vi "BSM Burst table save.vi"(6 "SN [ratio]":T1, 7 "Ex info":T4, 8 "error in":errorcluster caption="エラー入力", 9 "BC1":cluster{"B region#":i32, "Date":string}, 10 "BS Path":T2, 11 "Table CP":T3) -> (0 "error out":errorcluster caption="エラー出力", 2 "Table Tag":T5, 3 "Table CV":T6)   [LabVIEW 2018]
panel:
  out "SN":string[](array[string])
  out "Mx Intensity level [pA]":dbl
  out "BL Level [pA]":dbl
  out "Signal Intensity [pA]":dbl
  out "S/N ratio":dbl
  out "BS_E Time Table Path":path
  out "BS_E Signal Table Path":path
  out "BS_E CP Table Path":path
  out "Signal Tag":string[](array[string])
  out "Time Profile A Table":string[][](table) caption="Time A Table"
  out "CP Profile A Table":string[][](table) caption="CP A Table"
  out "Signal Profile A Table":string[][](table) caption="S Table"
  out "サブセット削除後の配列":string[](array[string])
  out "Level Composition":string[](array[string])
  out "Base Ex info array":string[](array[string])
  out "Time Profile Table":string[][](table) caption="Time Table"
  out "CP Profile Table":string[][](table) caption="CP Table"
  out "Signal Profile Table":string[][](table) caption="S Table"
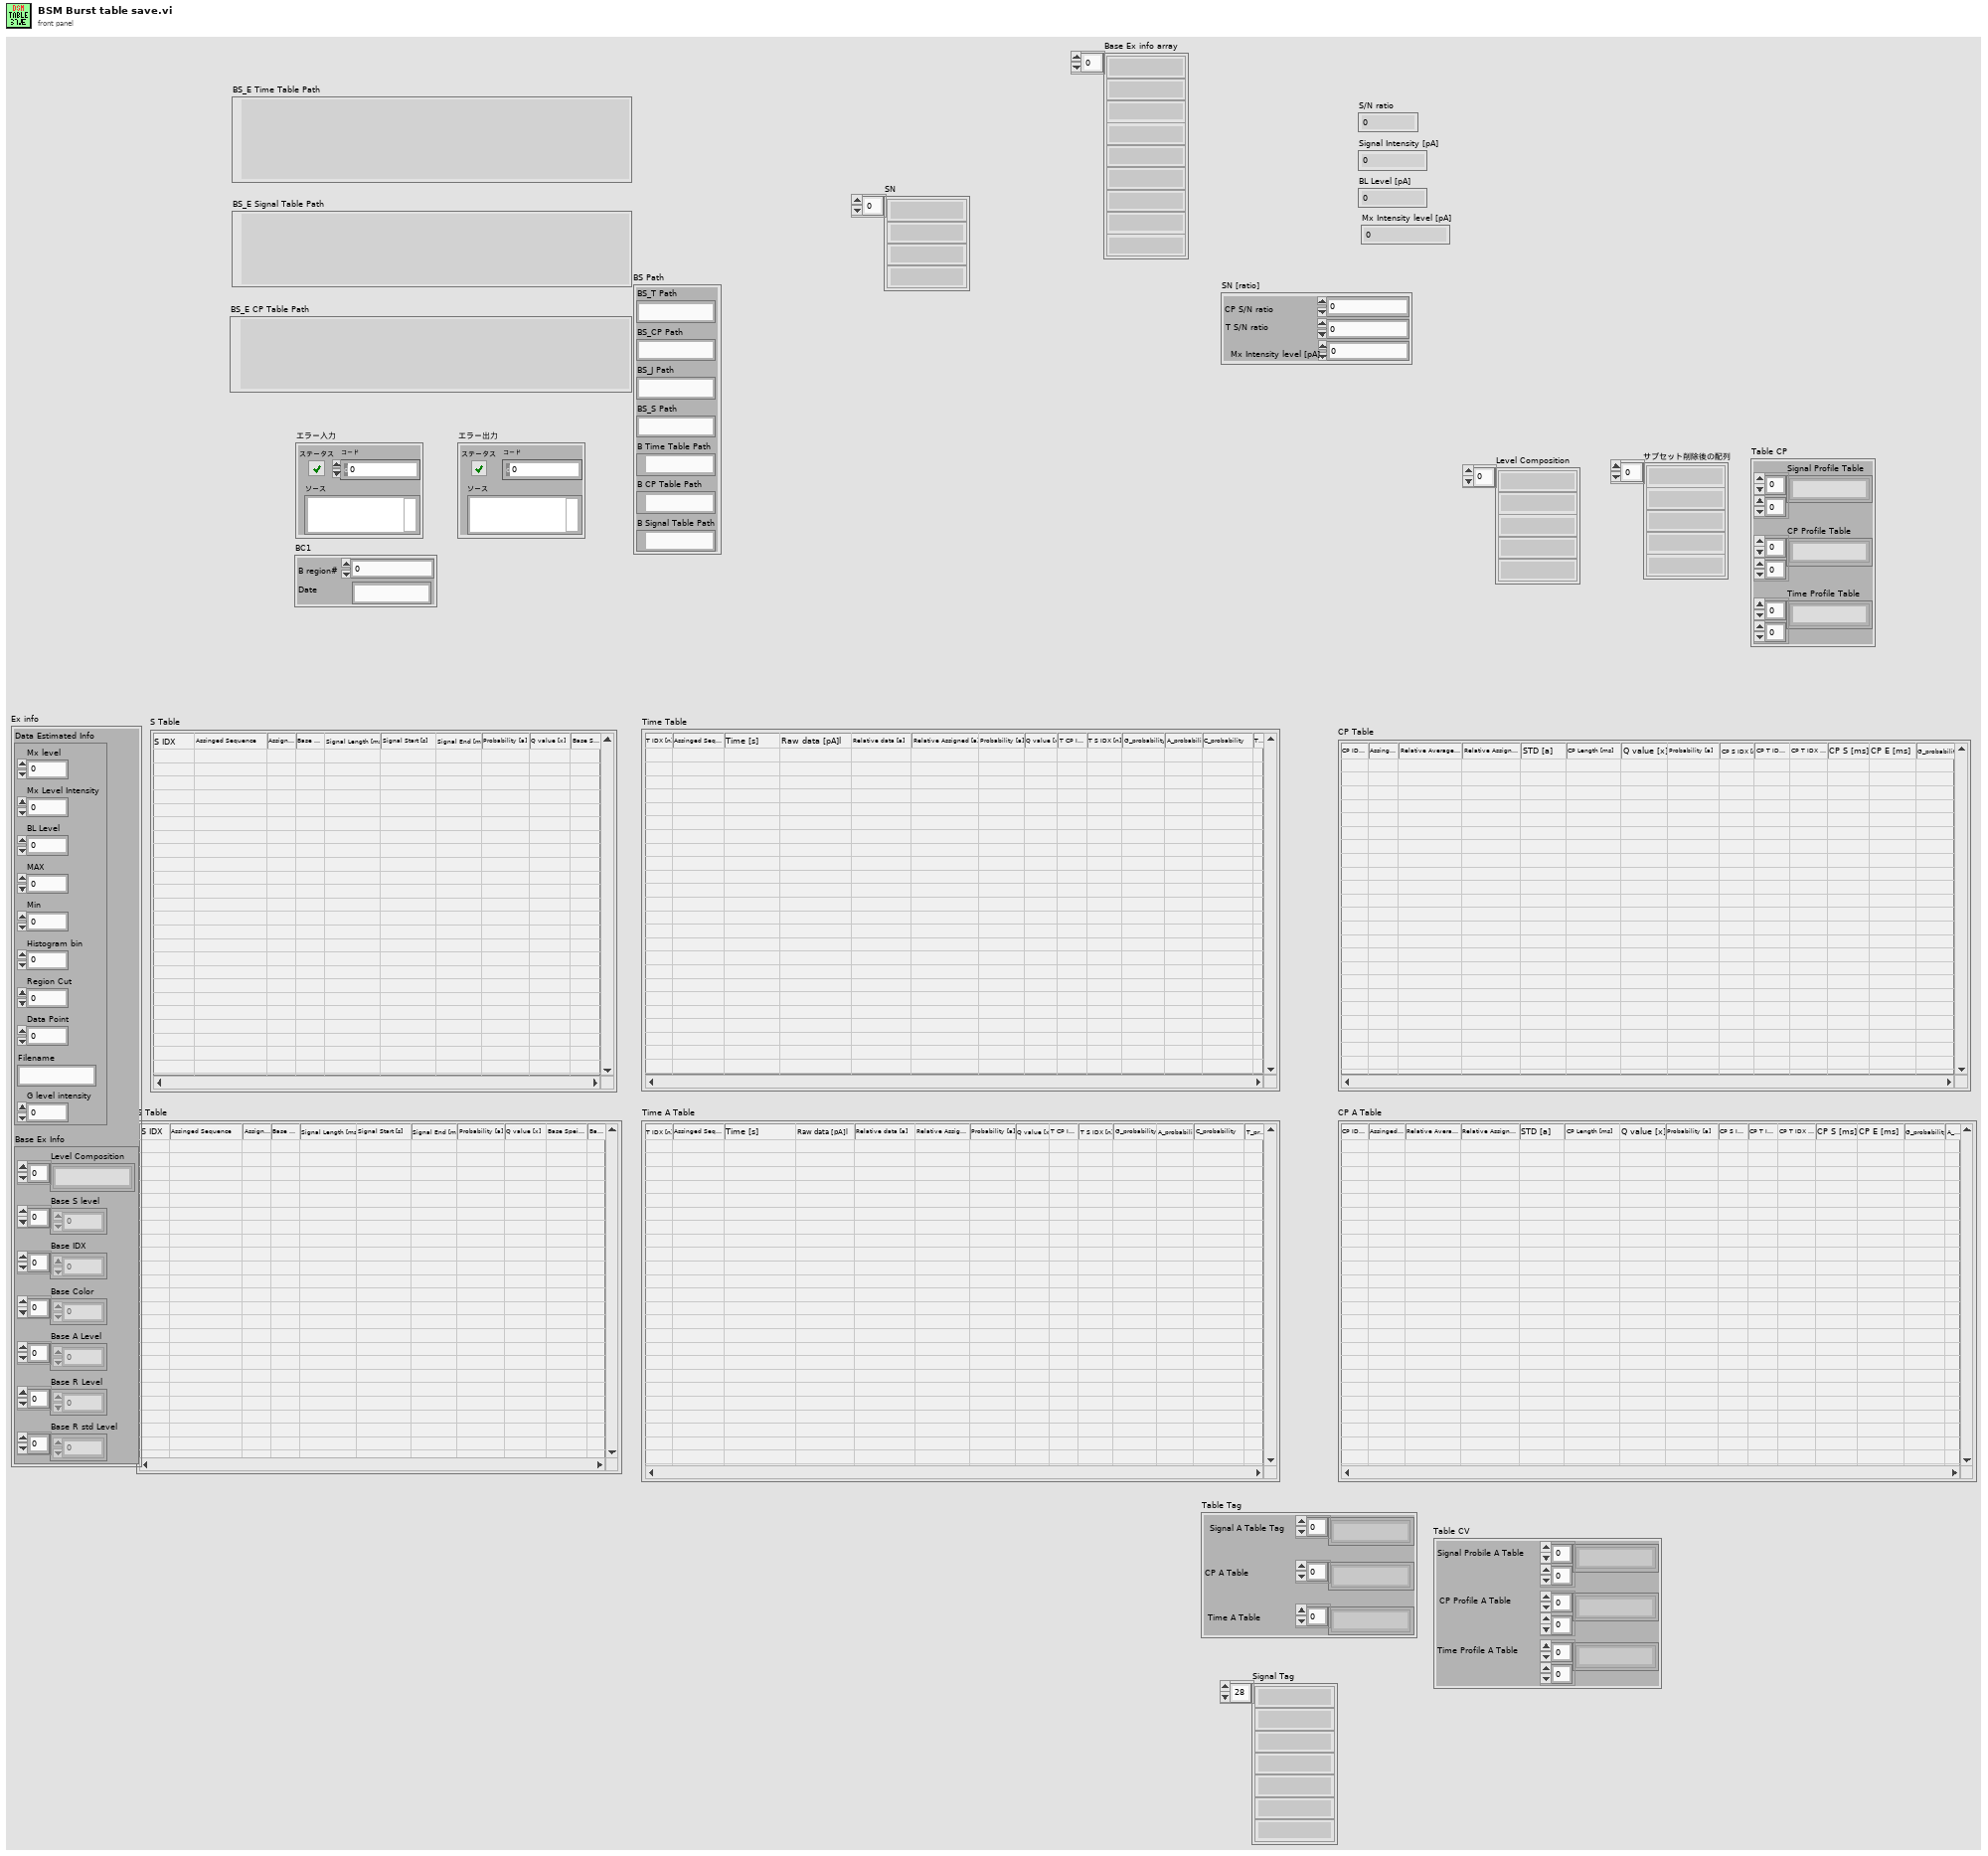
[diagram p1: front panel]
types:
  T1 = cluster{"CP S/N ratio":dbl, "T S/N ratio":dbl, "Mx Intensity level [pA]":dbl}
  T2 = cluster{"BS_T Path":string, "BS_CP Path":string, "BS_J Path":string, "BS_S Path":string, "B Time Table Path":path, "B CP Table Path":path, "B Signal Table Path":path}
  T3 = cluster{"Signal Profile Table":string[][], "CP Profile Table":string[][], "Time Profile Table":string[][]}
  T4 = cluster{"Data Estimated Info":cluster{"Mx level":dbl, "Mx Level Intensity":dbl, "BL Level":dbl, "MAX":dbl, "Min":dbl, "Histogram bin":dbl, "Region Cut":dbl, "Data Point":i32, "Filename":string, "G level intensity":dbl}, "Base Ex Info":cluster{"Level Composition":string[], "Base S level":dbl[], "Base IDX":i32[], "Base Color":u32[], "Base A Level":dbl[], "Base R Level":dbl[], "Base R std Level":dbl[]}}
  T5 = cluster{"Signal A Table Tag":string[], "CP A Table":string[], "Time A Table":string[]}
  T6 = cluster{"Signal Probile A Table":string[][], "CP Profile A Table":string[][], "Time Profile A Table":string[][]}
  T7 = enum16{"open", "replace", "create", "open or create", "replace or create", "replace or create with confirmation"}
  T8 = cluster{"Mx level":dbl, "Mx Level Intensity":dbl, "BL Level":dbl, "MAX":dbl, "Min":dbl, "Histogram bin":dbl, "Region Cut":dbl, "Data Point":i32, "Filename":string, "G level intensity":dbl}
  T9 = cluster{"Level Composition":string[], "Base S level":dbl[], "Base IDX":i32[], "Base Color":u32[], "Base A Level":dbl[], "Base R Level":dbl[], "Base R std Level":dbl[]}
  T10 = cluster{"行ヘッダ文字列[]":string[], "行ヘッダ文字列[]":string[], "行ヘッダ文字列[]":string[]}
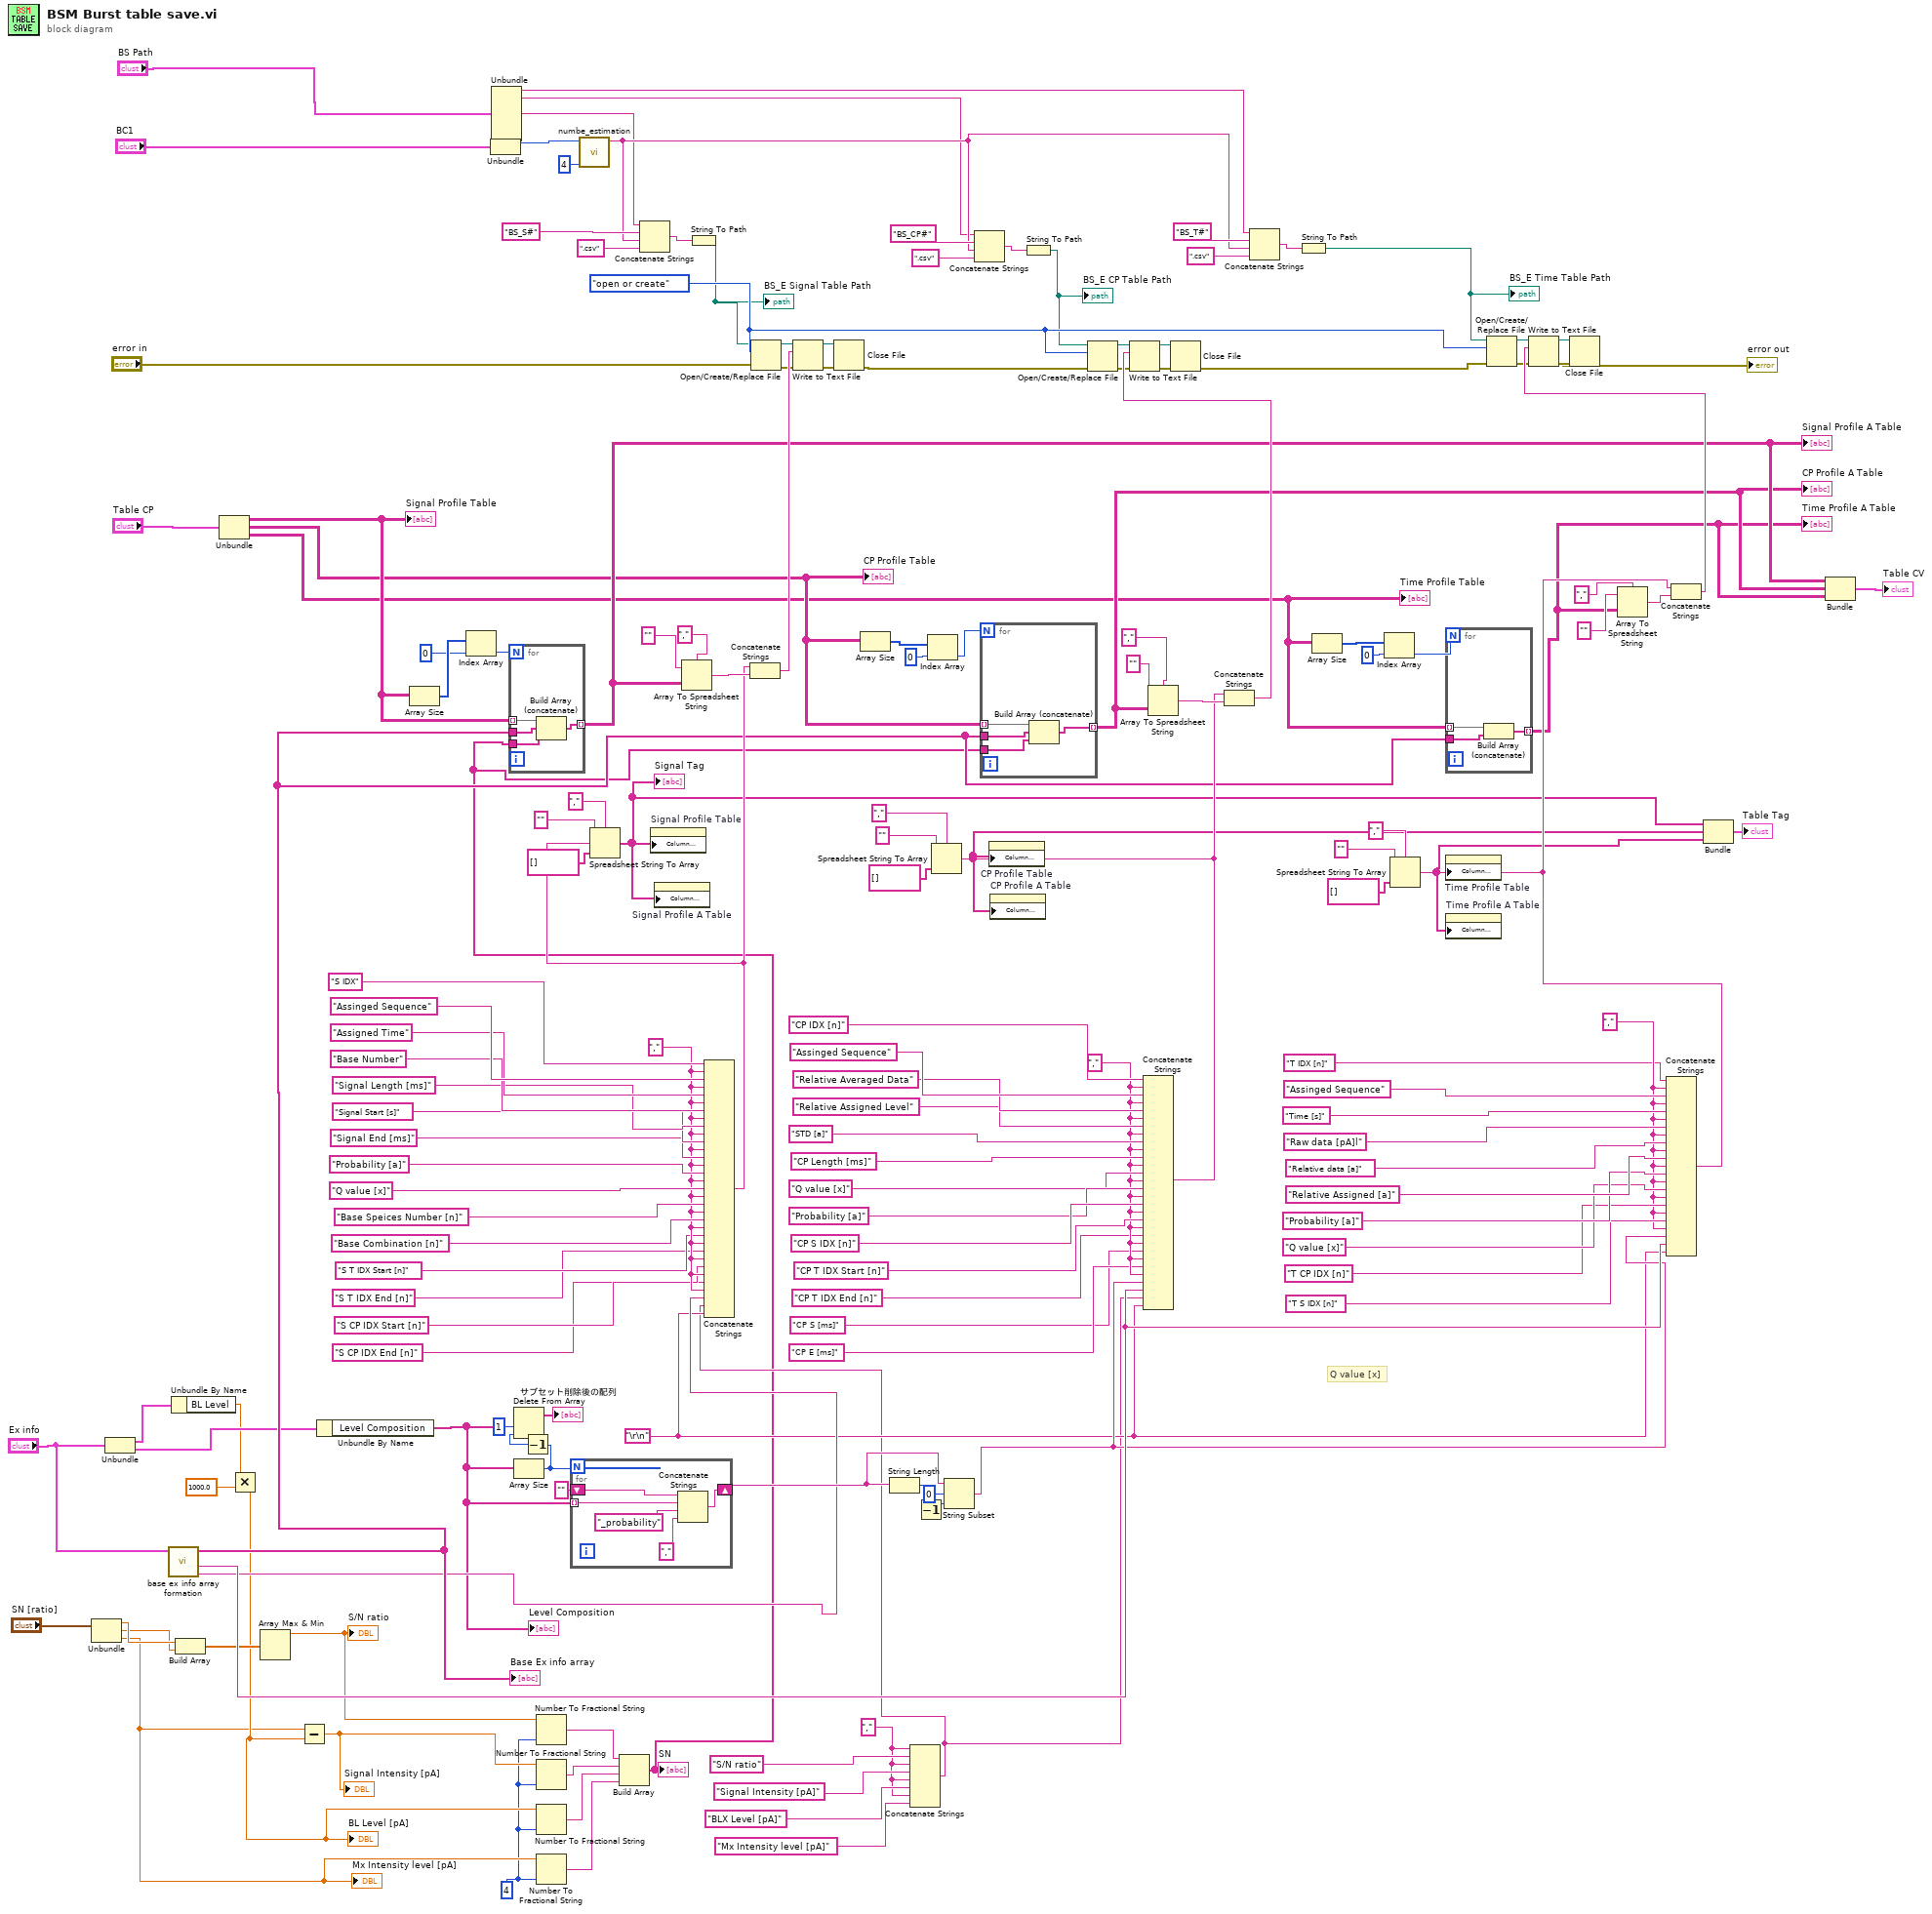
[diagram p0: block diagram]
diagram:
  w4 = "," ("デリミタ（タブ）")
  w13 = i16 4 ("精度（6）")
  w73 = T7."open or create" ("操作（0:open）")
  w68 = "," ("デリミタ（タブ）")
  w63 = "," ("デリミタ（タブ）")
  w59 = "," ("デリミタ（タブ）")
  w3 = "\r\n"
  # "Q value [x]"
  n1 = Unbundle("SN [ratio]") -> ("CP S/N ratio"=w22:dbl, "T S/N ratio"=w21:dbl, "Mx Intensity level [pA]"=w14:dbl)
  "Mx Intensity level [pA]" <- w14
  n2 = Unbundle("Ex info") -> ("Data Estimated Info"=w24:T8, "Base Ex Info"=w26:T9)
  n3 = call "base ex info array formation.vi"("Ex info"="Ex info") -> ("Tag"=w54:string, "Tag 2"=w65:string, "Base Ex info array"=w95:string[])  [unwired: 8 in]
  "Base Ex info array" <- w95
  n4 = Unbundle By Name(w24) -> ("BL Level"=w19:dbl)
  n5 = Build Array(w22, w21) -> (w20:dbl[])
  n6 = Unbundle("Table CP") -> ("Signal Profile Table"=w33:string[][], "CP Profile Table"=w32:string[][], "Time Profile Table"=w31:string[][])
  "Signal Profile Table" <- w33
  "CP Profile Table" <- w32
  "Time Profile Table" <- w31
  n7 = Multiply(x=w19, y=1000.0) -> (x*y=w15:dbl)
  "BL Level [pA]" <- w15
  n8 = Array Max & Min(array=w20) -> (max value=w17:dbl)  [unwired: 3 out]
  "S/N ratio" <- w17
  n9 = Subtract(x=w14, y=w15) -> (x-y=w16:dbl)
  "Signal Intensity [pA]" <- w16
  n10 = Unbundle By Name(w26) -> ("Level Composition"=w25:string[])
  "Level Composition" <- w25
  n11 = Array Size(array=w33) -> (size(s)=w107:i32[])
  n12 = Index Array(array=w107, index=0 ("指標")) -> (element=w105:i32)
  n13 = Unbundle("BC1") -> ("B region#"=w49:i32)  [unwired: 1 out]
  n14 = Unbundle("BS Path") -> ("BS_T Path"=w27:string, "BS_CP Path"=w30:string, "BS_S Path"=w28:string)  [unwired: 4 out]
  n15 = Array Size(array=w25) -> (size(s)=w127:i32)
  n16 = Decrement(x=w127) -> (x-1=w128:i32)
  n17 = Delete From Array(array=w25, length=1 ("長さ"), index=w128) -> (array with subset deleted=→"サブセット削除後の配列":string[])  [unwired: 1 out]
  n18 = Number To Fractional String(number=w17, precision (6)=w13) -> (F-format string=w12:string)  [unwired: 2 in]
  n19 = Number To Fractional String(number=w16, precision (6)=w13) -> (F-format string=w11:string)  [unwired: 2 in]
  n20 = Number To Fractional String(number=w15, precision (6)=w13) -> (F-format string=w10:string)  [unwired: 2 in]
  n21 = Number To Fractional String(number=w14, precision (6)=w13) -> (F-format string=w9:string)  [unwired: 2 in]
  n22 = for {
    N: w127 -> [_]
    tunnel: w25 -> [w168] mode=indexing
    shift-right: [w167] -> w122
    shift-left: "" -> [w166]
    n23 = Concatenate Strings(w166, w168, "_probability" ("文字列"), "," ("デリミタ（タブ）")) -> (w167:string)
  }
  n24 = call "numbe_estimation.vi"("桁数"=4, "数値"=w49) -> ("数値文字列"=w37:string)  [unwired: 9 in]
  n25 = Build Array(w12, w11, w10, w9) -> (w1:string[])
  "SN" <- w1
  n26 = for {
    N: w105 -> [_]
    tunnel: w33 -> [w172] mode=indexing
    tunnel: w95 -> [w171]
    tunnel: [w170] -> w94 mode=indexing
    tunnel: w1 -> [w169]
    n27 = Build Array (concatenate)(w172, w171, w169) -> (w170:string[])
  }
  "Signal Profile A Table" <- w94
  n28 = Concatenate Strings(w28, "BS_S#" ("文字列"), w37, ".csv" ("文字列")) -> (w46:string)
  n29 = Array To Spreadsheet String(delimiter (Tab)="," ("デリミタ（タブ）"), array=w94, 3:"" ("形式文字列")) -> (spreadsheet string=w161:string)
  n30 = String To Path(string=w46) -> (path=w45:path)
  "BS_E Signal Table Path" <- w45
  n31 = Open/Create/Replace File(file path (use dialog)=w45, error in="error in", operation (0:open)=w73) -> (refnum out=w81:refnum<file>, error out=w82:errorcluster)  [unwired: 3 in, 1 out]
  n32 = Array Size(array=w32) -> (size(s)=w100:i32[])
  n33 = String Length(string=w122) -> (length=w124:i32)
  n34 = Concatenate Strings(w4, "S/N ratio" ("書き込みバッファ"), w4, "Signal Intensity [pA]" ("書き込みバッファ"), w4, "BLX Level [pA]" ("書き込みバッファ"), w4, "Mx Intensity level [pA]" ("書き込みバッファ")) -> (w2:string)
  n35 = Concatenate Strings("S IDX" ("文字列"), w59, "Assinged Sequence" ("書き込みバッファ"), w59, "Assigned Time" ("書き込みバッファ"), w59, "Base Number" ("書き込みバッファ"), w59, "Signal Length [ms]" ("書き込みバッファ"), w59, "Signal Start [s]" ("書き込みバッファ"), w59, "Signal End [ms]" ("書き込みバッファ"), w59, "Probability [a]" ("書き込みバッファ"), w59, "Q value [x]" ("書き込みバッファ"), w59, "Base Speices Number [n]" ("書き込みバッファ"), w59, "Base Combination [n]" ("書き込みバッファ"), w59, "S T IDX Start [n]" ("書き込みバッファ"), w59, "S T IDX End [n]" ("書き込みバッファ"), w59, "S CP IDX Start [n]" ("書き込みバッファ"), w59, "S CP IDX End [n]" ("書き込みバッファ"), w59, w54, w2, w3) -> (w117:string)
  n36 = Spreadsheet String To Array(delimiter (Tab)="," ("デリミタ（タブ）"), format string="" ("形式文字列"), spreadsheet string=w117, array type (2D Dbl)=string[] [] ("行ヘッダ文字列[]")) -> (array=w90:string[])
  "Signal Tag" <- w90
  n37 = property on="Signal Profile Table" class="Tbl (strict)"("Column Headers[]"=w90) -> ()  [unwired: 2 in, 2 out]
  n38 = property on="Signal Profile A Table" class="Tbl (strict)"("Column Headers[]"=w90) -> ()  [unwired: 2 in, 2 out]
  n39 = Concatenate Strings(w117, w161) -> (w146:string)
  n40 = Write to Text File(file (use dialog)=w81, text=w146, error in=w82) -> (refnum out=w80:refnum<file>, error out=w79:errorcluster)  [unwired: 1 in, 1 out]
  n41 = Close File(refnum=w80, error in=w79) -> (error out=w78:errorcluster)  [unwired: 1 out]
  n42 = Decrement(x=w124) -> (x-1=w123:i32)
  n43 = Index Array(array=w100, index=0 ("指標")) -> (element=w98:i32)
  n44 = String Subset(string=w122, offset (0)=0 ("オフセット（0）"), length (rest)=w123) -> (substring=w64:string)
  n45 = Concatenate Strings(w30, "BS_CP#" ("文字列"), w37, ".csv" ("文字列")) -> (w42:string)
  n46 = for {
    N: w98 -> [_]
    tunnel: w32 -> [w176] mode=indexing
    tunnel: w95 -> [w175]
    tunnel: [w174] -> w93 mode=indexing
    tunnel: w1 -> [w173]
    n47 = Build Array (concatenate)(w176, w175, w173) -> (w174:string[])
  }
  "CP Profile A Table" <- w93
  n48 = String To Path(string=w42) -> (path=w41:path)
  "BS_E CP Table Path" <- w41
  n49 = Open/Create/Replace File(file path (use dialog)=w41, error in=w78, operation (0:open)=w73) -> (refnum out=w85:refnum<file>, error out=w86:errorcluster)  [unwired: 3 in, 1 out]
  n50 = Concatenate Strings("CP IDX [n]" ("文字列"), w63, "Assinged Sequence" ("書き込みバッファ"), w63, "Relative Averaged Data" ("書き込みバッファ"), w63, "Relative Assigned Level" ("書き込みバッファ"), w63, "STD [a]" ("書き込みバッファ"), w63, "CP Length [ms]" ("書き込みバッファ"), w63, "Q value [x]" ("書き込みバッファ"), w63, "Probability [a]" ("書き込みバッファ"), w63, "CP S IDX [n]" ("書き込みバッファ"), w63, "CP T IDX Start [n]" ("書き込みバッファ"), w63, "CP T IDX End [n]" ("書き込みバッファ"), w63, "CP S [ms]" ("書き込みバッファ"), w63, "CP E [ms]" ("書き込みバッファ"), w63, w64, w65, w2, w3) -> (w110:string)
  n51 = Spreadsheet String To Array(delimiter (Tab)="," ("デリミタ（タブ）"), format string="" ("形式文字列"), spreadsheet string=w110, array type (2D Dbl)=string[] [] ("行ヘッダ文字列[]")) -> (array=w89:string[])
  n52 = property on="CP Profile Table" class="Tbl (strict)"("Column Headers[]"=w89) -> ()  [unwired: 2 in, 2 out]
  n53 = property on="CP Profile A Table" class="Tbl (strict)"("Column Headers[]"=w89) -> ()  [unwired: 2 in, 2 out]
  n54 = Array To Spreadsheet String(delimiter (Tab)="," ("デリミタ（タブ）"), array=w93, 3:"" ("形式文字列")) -> (spreadsheet string=w150:string)
  n55 = Concatenate Strings(w110, w150) -> (w121:string)
  n56 = Write to Text File(file (use dialog)=w85, text=w121, error in=w86) -> (refnum out=w84:refnum<file>, error out=w83:errorcluster)  [unwired: 1 in, 1 out]
  n57 = Close File(refnum=w84, error in=w83) -> (error out=w72:errorcluster)  [unwired: 1 out]
  n58 = Concatenate Strings(w27, "BS_T#" ("文字列"), w37, ".csv" ("文字列")) -> (w38:string)
  n59 = String To Path(string=w38) -> (path=w36:path)
  "BS_E Time Table Path" <- w36
  n60 = Array Size(array=w31) -> (size(s)=w97:i32[])
  n61 = Index Array(array=w97, index=0 ("指標")) -> (element=w35:i32)
  n62 = for {
    N: w35 -> [_]
    tunnel: w31 -> [w179] mode=indexing
    tunnel: w95 -> [w178]
    tunnel: [w177] -> w92 mode=indexing
    n63 = Build Array (concatenate)(w179, w178) -> (w177:string[])
  }
  "Time Profile A Table" <- w92
  n64 = Open/Create/Replace File(file path (use dialog)=w36, error in=w72, operation (0:open)=w73) -> (refnum out=w76:refnum<file>, error out=w77:errorcluster)  [unwired: 3 in, 1 out]
  n65 = Array To Spreadsheet String(delimiter (Tab)="," ("デリミタ（タブ）"), array=w92, 3:"" ("形式文字列")) -> (spreadsheet string=w147:string)
  n66 = Concatenate Strings("T IDX [n]" ("文字列"), w68, "Assinged Sequence" ("書き込みバッファ"), w68, "Time [s]" ("書き込みバッファ"), w68, "Raw data [pA]l" ("書き込みバッファ"), w68, "Relative data [a]" ("書き込みバッファ"), w68, "Relative Assigned [a]" ("書き込みバッファ"), w68, "Probability [a]" ("書き込みバッファ"), w68, "Q value [x]" ("書き込みバッファ"), w68, "T CP IDX [n]" ("書き込みバッファ"), w68, "T S IDX [n]" ("書き込みバッファ"), w68, w64, w65, w3) -> (w109:string)
  n67 = Spreadsheet String To Array(delimiter (Tab)="," ("デリミタ（タブ）"), format string="" ("形式文字列"), spreadsheet string=w109, array type (2D Dbl)=string[] [] ("行ヘッダ文字列[]")) -> (array=w88:string[])
  n68 = property on="Time Profile Table" class="Tbl (strict)"("Column Headers[]"=w88) -> ()  [unwired: 2 in, 2 out]
  n69 = property on="Time Profile A Table" class="Tbl (strict)"("Column Headers[]"=w88) -> ()  [unwired: 2 in, 2 out]
  n70 = Concatenate Strings(w109, w147) -> (w132:string)
  n71 = Write to Text File(file (use dialog)=w76, text=w132, error in=w77) -> (refnum out=w75:refnum<file>, error out=w74:errorcluster)  [unwired: 1 in, 1 out]
  n72 = Close File(refnum=w75, error in=w74) -> (error out=→"error out":errorcluster)  [unwired: 1 out]
  n73 = Bundle("行ヘッダ文字列[]"=w90, "行ヘッダ文字列[]"=w89, "行ヘッダ文字列[]"=w88) -> (→"Table Tag":T10)  [unwired: 1 in]
  n74 = Bundle(w94, w93, w92) -> (→"Table CV":cluster{string[][], string[][], string[][]})  [unwired: 1 in]
